vi "recovery_pulses__12610e41b4.vi"(6 "offset (sec)":dbl=0.005, 7 "trigger voltage":dbl=3.8 format="%0.2f", 8 "edge":i32(ring)=10171 items=["Rising"=10280, "Falling"=10171], 9 "recovery points per half period":dbl=10.0, 10 "Pulse high time (s)":dbl=0.0001, 11 "frequency":dbl) -> (3 "output array":cluster{dbl, dbl}[](array[cluster]))   [LabVIEW 2023]
uses:
  <vilib>/Utility/error.llb/DialogType.ctl
  <vilib>/DAQmx/write.llb/DAQmx Write (Analog DBL 1Chan 1Samp).vi
  <vilib>/DAQmx/write.llb/DAQmx Write (Counter 1D Time 1Chan NSamp).vi
  <vilib>/DAQmx/create/channels.llb/DAQmx Create Channel (AO-Voltage-Basic).vi
  <vilib>/DAQmx/miscellaneous.llb/DAQmx Fill In Error Info.vi
  <vilib>/DAQmx/create/channels.llb/DAQmx Create Channel (CO-Pulse Generation-Time).vi
  <vilib>/DAQmx/configure/trigger.llb/DAQmx Start Trigger (Digital Edge).vi
  <vilib>/DAQmx/configure/timing.llb/DAQmx Timing (Implicit).vi
  <resource>/objmgr/daqmx.rc
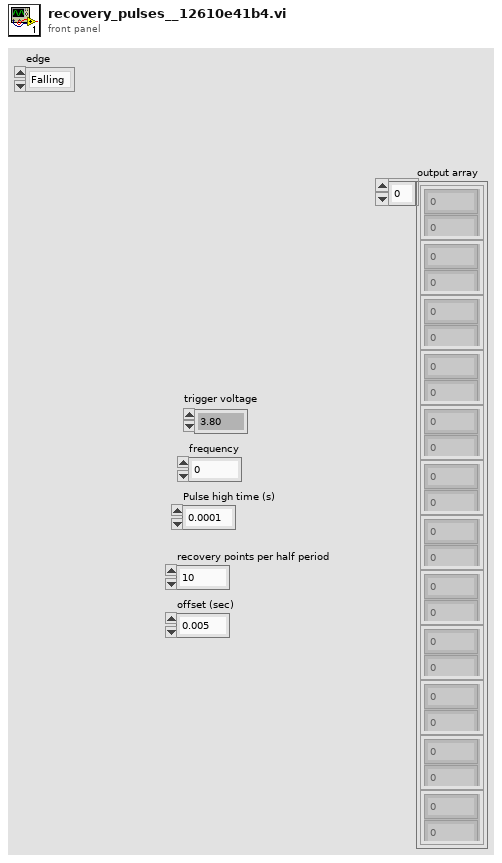
[diagram p1: front panel]
types:
  T1 = typedef "DialogType.ctl" = u16
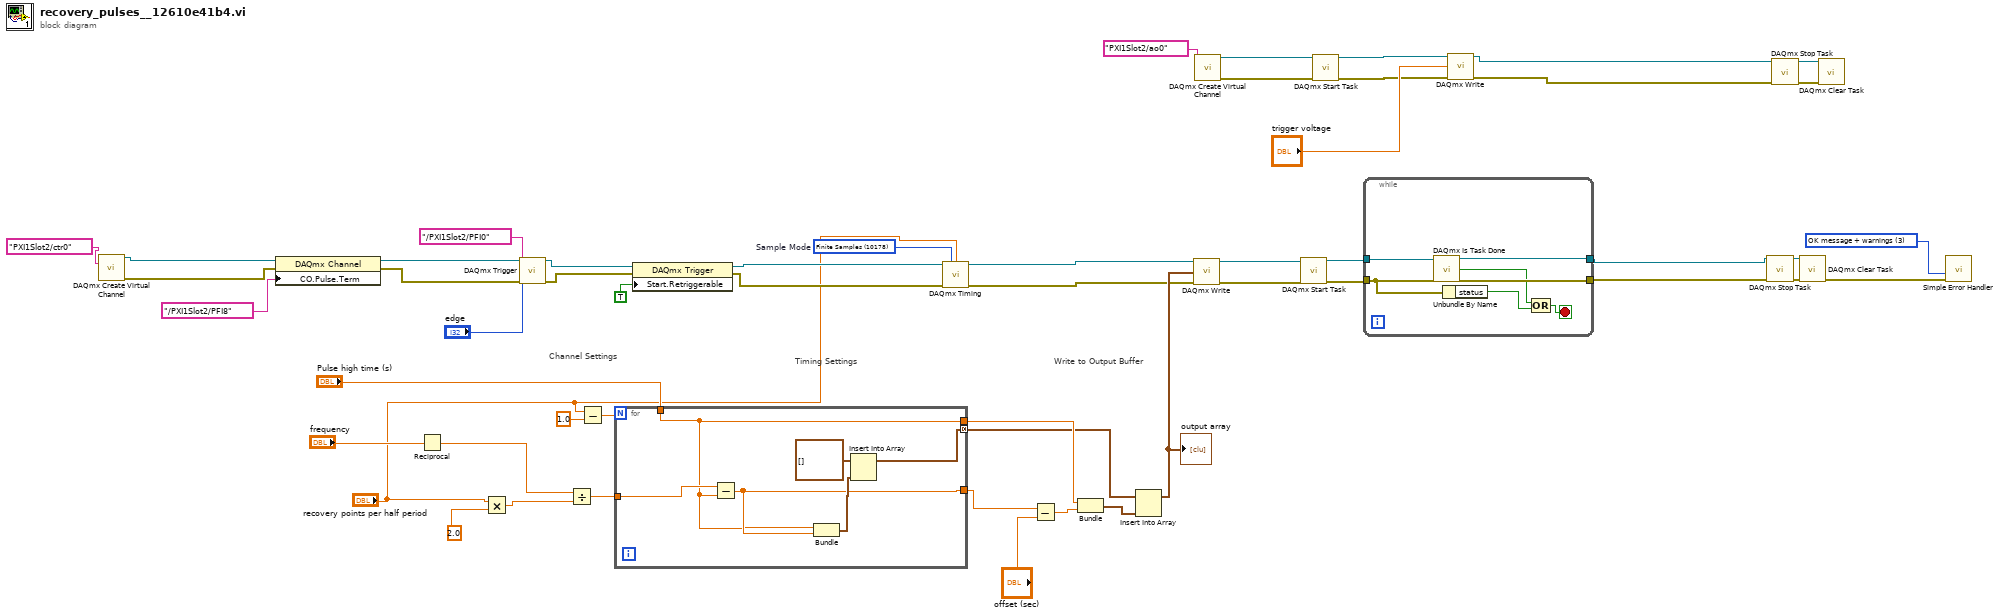
[diagram p0: block diagram]
diagram:
  w49 = 10178 items=["Finite Samples"=10178, "Continuous Samples"=10123, "Hardware Timed Single Point"=12522]  # Sample Mode
  w15 = T1 3 items=["no dialog", "OK message", "continue or stop message", "OK message + warnings", "continue/stop + warnings"] ("type of dialog (OK msg:1)")
  # "Write to Output Buffer"
  # "Timing Settings"
  # "Channel Settings"
  n1 = call-poly <vilib>:"DAQmx Create Virtual Channel.vi"("counter"=tag "PXI1Slot2/ctr0") -> ("task out"=w51:refnum<k21>, "error out"=w52:errorcluster)  [unwired: 13 in]
  n2 = property class="DAQmx Channel"(reference=w51, error in=w52, "CO.Pulse.Term"=tag "/PXI1Slot2/PFI8") -> (reference out=w16:refnum<k21>, error out=w17:errorcluster)
  n3 = Reciprocal(x="frequency") -> (1/x=w46:dbl)
  n4 = Multiply(x="recovery points per half period", y=2.0) -> (x*y=w1:dbl)
  n5 = call-poly <vilib>:"DAQmx Trigger.vi"("task/channels in"=w16, "source"=tag "/PXI1Slot2/PFI0", "edge"="edge", "error in"=w17) -> ("task out"=w19:refnum<k21>, "error out"=w20:errorcluster)  [unwired: 10 in]
  n6 = Divide(x=w46, y=w1) -> (x/y=w22:dbl)
  n7 = Subtract(x="recovery points per half period", y=1.0) -> (x-y=w23:dbl)
  n8 = for {
    N: w23 -> [_]
    tunnel: [w56] -> w27 mode=concatenating
    tunnel: w22 -> [w58]
    tunnel: [w54] -> w25
    tunnel: [w53] -> w28
    tunnel: "Pulse high time (s)" -> [w53]
    n9 = Subtract(x=w58, y=w53) -> (x-y=w54:dbl)
    n10 = Bundle("Pulse high time (s)"=w53, w54) -> (w57:cluster{"Pulse high time (s)":dbl, dbl})  [unwired: 1 in]
    n11 = Insert Into Array(array=cluster{dbl, dbl}[] [], new element=w57) -> (w56:cluster{dbl, dbl}[])  [unwired: 1 in]
  }
  n12 = property class="DAQmx Trigger"(reference=w19, error in=w20, "Start.Retriggerable"=TRUE) -> (reference out=w42:refnum<k21>, error out=w43:errorcluster)
  n13 = call-poly <vilib>:"DAQmx Timing.vi"("task/channels in"=w42, "sample mode"=w49, "samples per channel"="recovery points per half period", "error in"=w43) -> ("task out"=w12:refnum<k21>, "error out"=w11:errorcluster)  [unwired: 10 in]
  n14 = Subtract(x=w25, y="offset (sec)") -> (x-y=w26:dbl)
  n15 = Bundle("Pulse high time (s)"=w28, w26) -> (w29:cluster{"Pulse high time (s)":dbl, dbl})  [unwired: 1 in]
  n16 = Insert Into Array(array=w27, new element=w29) -> (w30:cluster{dbl, dbl}[])  [unwired: 1 in]
  "output array" <- w30
  n17 = call-poly <vilib>:"DAQmx Write.vi"("task/channels in"=w12, "data"=w30, "error in"=w11) -> ("task out"=w47:refnum<k21>, "error out"=w48:errorcluster)  [unwired: 10 in, 1 out]
  n18 = call-poly <vilib>:"DAQmx Create Virtual Channel.vi"("physical channels"=tag "PXI1Slot2/ao0") -> ("task out"=w33:refnum<k21>, "error out"=w34:errorcluster)  [unwired: 13 in]
  n19 = call <vilib>:"DAQmx Start Task.vi"("task/channels in"=w47, "error in"=w48) -> ("task out"=w8:refnum<k21>, "error out"=w7:errorcluster)  [unwired: 12 in]
  n20 = call <vilib>:"DAQmx Start Task.vi"("task/channels in"=w33, "error in"=w34) -> ("task out"=w35:refnum<k21>, "error out"=w36:errorcluster)  [unwired: 12 in]
  n21 = while {
    tunnel: w8 -> [w63]
    tunnel: w7 -> [w60]
    tunnel: [w61] -> w5
    tunnel: [w62] -> w6
    stop <- w65 stop-if-true
    n22 = call <vilib>:"DAQmx Is Task Done.vi"("task/channels in"=w63, "error in"=w60) -> ("task out"=w62:refnum<k21>, "task done?"=w59:bool, "error out"=w61:errorcluster)  [unwired: 11 in]
    n23 = Unbundle By Name(w60) -> ("status"=w64:bool)
    n24 = Compound Arithmetic op=OR(w59, w64) -> (w65:bool)
  }
  n25 = call-poly <vilib>:"DAQmx Write.vi"("task/channels in"=w35, "data"="trigger voltage", "error in"=w36) -> ("task out"=w37:refnum<k21>, "error out"=w38:errorcluster)  [unwired: 10 in, 1 out]
  n26 = call <vilib>:"DAQmx Stop Task.vi"("task/channels in"=w6, "error in"=w5) -> ("task out"=w13:refnum<k21>, "error out"=w14:errorcluster)  [unwired: 12 in]
  n27 = call <vilib>:"DAQmx Stop Task.vi"("task/channels in"=w37, "error in"=w38) -> ("task out"=w39:refnum<k21>, "error out"=w40:errorcluster)  [unwired: 12 in]
  n28 = call <vilib>:"DAQmx Clear Task.vi"("task in"=w13, "error in"=w14) -> ("error out"=w10:errorcluster)  [unwired: 13 in]
  n29 = call <vilib>:"DAQmx Clear Task.vi"("task in"=w39, "error in"=w40) -> ()  [unwired: 13 in, 1 out]
  n30 = call <vilib>:"Simple Error Handler.vi"("type of dialog (OK msg:1)"=w15, "error in (no error)"=w10) -> ()  [unwired: 3 in, 5 out]
